vi "Own20261012_GetBooleanText.vi"() -> ()   [LabVIEW 2024]
panel:
  out "error out":errorcluster caption="错误输出"
  out "text":string
  in  "boolean_id":u32
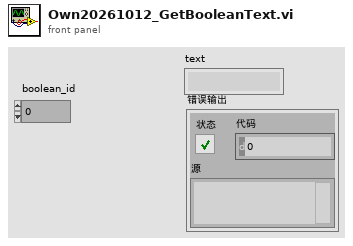
[diagram p1: front panel]
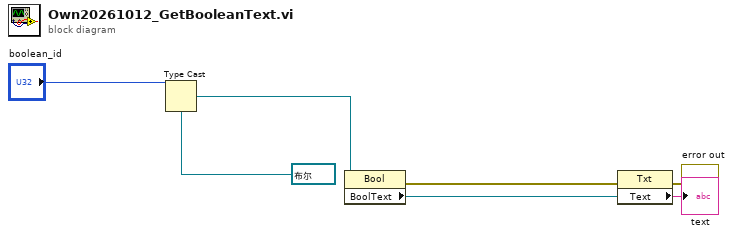
[diagram p0: block diagram]
diagram:
  n1 = Type Cast(type=refnum<vi> refnum ("引用"), x="boolean_id") -> (*(type *) &x=w5:refnum<vi>)
  n2 = property class="Bool"(reference=w5) -> (error out=w3:errorcluster, "BoolText"=w4:refnum<vi>)  [unwired: 1 in, 1 out]
  n3 = property class="Txt"(reference=w4, error in=w3) -> (error out=→"error out":errorcluster, "Text"=→"text":string)  [unwired: 1 out]
